vi "Add News.vi"(8 "direction":string, 9 "stocks":i32[](array[numeric]), 10 "headline":string, 11 "market":T1) -> (3 "market out":T1)   [LabVIEW 2020, in "Full Featured MCP Server.lvlib"]
doc: "Puts a news item at the top of the news list and keeps the latest 50 items. The item records the second it was published, so readers can compare prices before and after."
uses:
  Full Featured MCP Server.lvlib
  Market State.ctl
  News Item.ctl
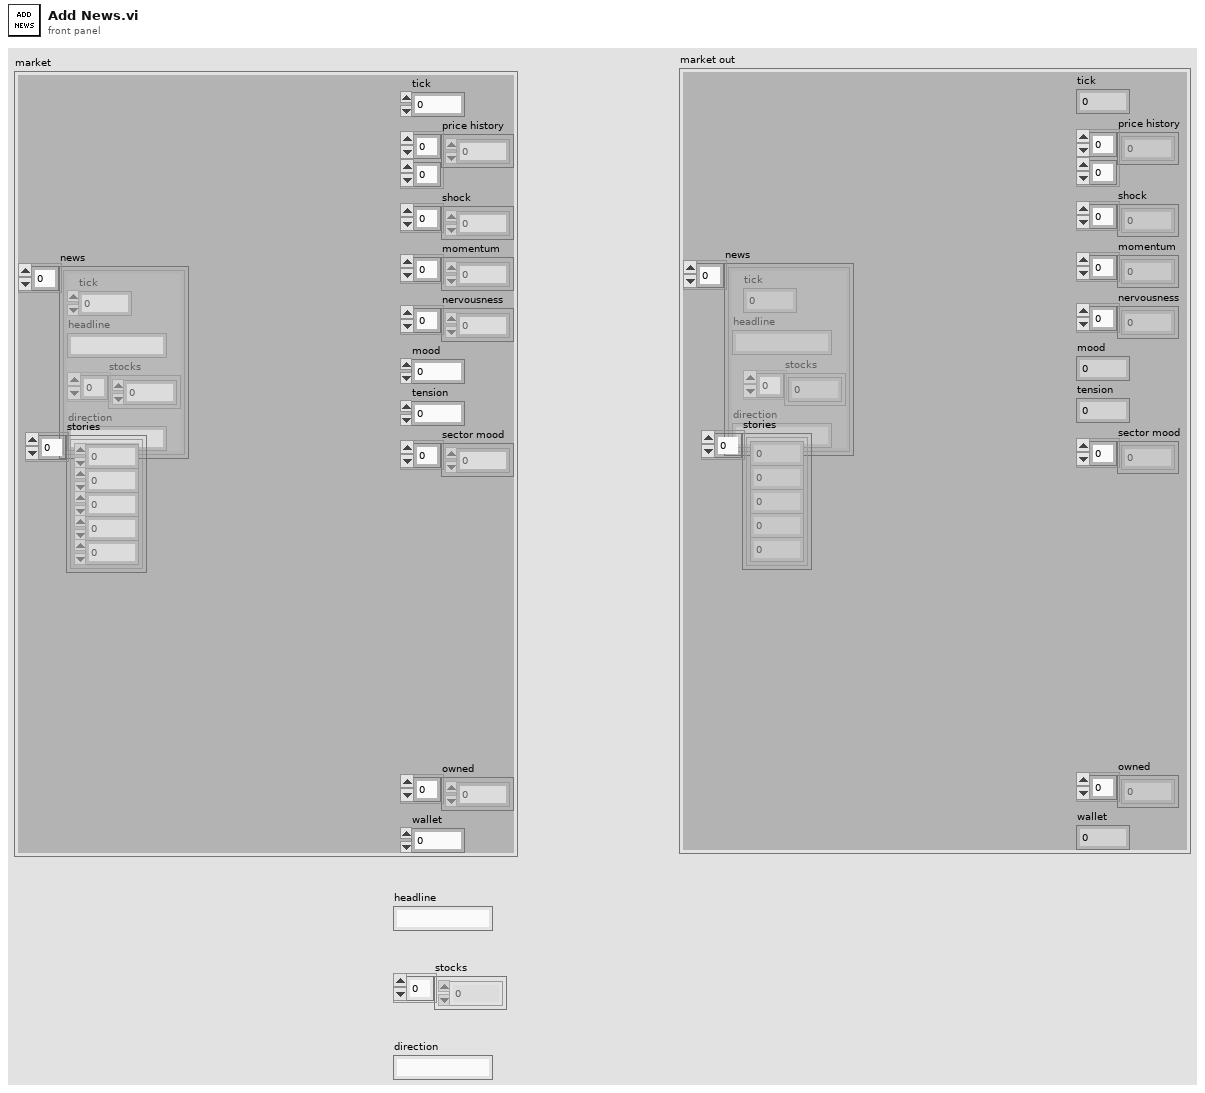
[diagram p1: front panel]
types:
  T1 = typedef "Full Featured MCP Server.lvlib/Market State.ctl" = cluster{"tick":i32, "price history":dbl[][], "shock":dbl[], "momentum":dbl[], "nervousness":dbl[], "mood":dbl, "tension":dbl, "sector mood":dbl[], "news":T2[], "stories":cluster{"arc":i32, "step":i32, "due":i32, "stock":i32, "other":i32}[], "owned":i32[], "wallet":dbl}
  T2 = typedef "Full Featured MCP Server.lvlib/News Item.ctl" = cluster{"tick":i32, "headline":string, "stocks":i32[], "direction":string}
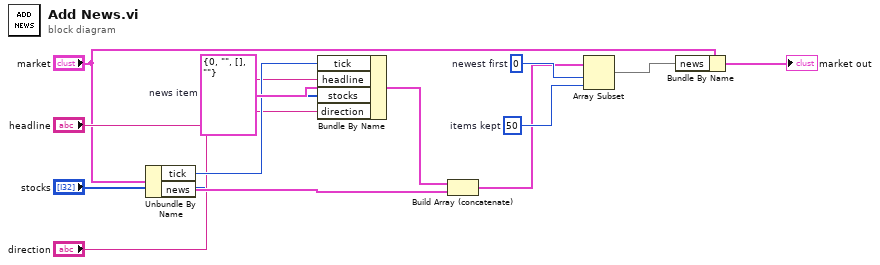
[diagram p0: block diagram]
diagram:
  w11 = 50  # items kept
  w10 = 0  # newest first
  w7 = T2 {"tick"=0, "headline"="", "stocks"=[], "direction"=""}  # news item
  n1 = Unbundle By Name("market") -> ("tick"=w5:i32, "news"=w6:T2[])
  n2 = Bundle By Name(cluster=w7, "tick"=w5, "headline"="headline", "stocks"="stocks", "direction"="direction") -> (w8:T2)
  n3 = Build Array (concatenate)(w8, w6) -> (w9:T2[])
  n4 = Array Subset(array=w9, index=w10, length=w11) -> (w12:T2[])
  n5 = Bundle By Name(cluster="market", "news"=w12) -> (→"market out":T1)
